vi "ReversedEngineering CreateStateTransationEdges.vi"(1 "GraphRefToAddNodesTo":refnum<class "Graph.lvclass">, 2 "StateDiagramReverseOptions":T1={"Clear All Current States"=TRUE, "UseMenuItem"=TRUE, "InsertArrayQueuedElementsVI"="", "Add Actions"=FALSE, "StateDiagramSerachActions"={"Action"=enum."NotTheseVIs", "VINames"=[], "LimitActions(VIs)"=10}, "AddCaseCommentsAsActions"=FALSE, "IgnoreStatesNotUsed"=FALSE, "CommentsSerachActions"={"MinimumTextLength"=0, "OnlyTopLeftComment"=FALSE, "CommentPrefix"=""}, "TransitionMode"=enum."Add to current transtion text", "ActionMode"=enum."Add to current action text"}, 3 "States":T5[](array[typedef]), 5 "error in (no error)":errorcluster, 7 "graphics":refnum<class "Graphics.lvclass">, 9 "grid":refnum<class "Grid.lvclass">) -> (19 "error out":errorcluster)   [LabVIEW 2020]
uses:
  <resource>/Framework/Providers/Open_GDS/UML/ReversedEngineering/ReversedEngineering StateMachineStateInfo.ctl
  <resource>/Framework/Providers/Open_GDS/UML/Graph_class/Graph.lvclass
  <resource>/Framework/Providers/Open_GDS/UML/Graphics_class/Graphics.lvclass
  <resource>/Framework/Providers/Open_GDS/UML/Grid_class/Grid.lvclass
  <resource>/Framework/Providers/Open_GDS/UML/ReversedEngineering/private/ReversedEngineering StateDiagramReverseOptions.ctl
  <resource>/Framework/Providers/Open_GDS/UML/ReversedEngineering/private/ReversedEngineering StateDiagramSerachActions.ctl
  <resource>/Framework/Providers/Open_GDS/UML/ReversedEngineering/ReversedEngineering StateAnalyseVIAction.ctl
  <resource>/Framework/Providers/Open_GDS/UML/ReversedEngineering/private/ReversedEngineering StateDiagramCommentSearchType.ctl
  <resource>/Framework/Providers/Open_GDS/UML/AbstractEdge_class/AbstractEdge.lvclass
  <resource>/Framework/Providers/Open_GDS/UML/StateNode_class/StateNode.lvclass
  <resource>/Framework/Providers/Open_GDS/UML/StateTransitionEdge_class/StateTransitionEdge.lvclass
  C:/Program Files (x86)/National Instruments/LabVIEW 2020/resource/Framework/Providers/Open_GDS/UML/AbstractEdge_class/AbstractEdge.lvclass
  <resource>/Framework/Providers/Open_GDS/UML/MultiLineString_class/MultiLineString.lvclass
  <resource>/Framework/Providers/Open_GDS/UML/AbstractNode_class/AbstractNode.lvclass
  <resource>/Framework/Providers/Open_GDS/UML/StateReverse_class/StateReverse.lvclass
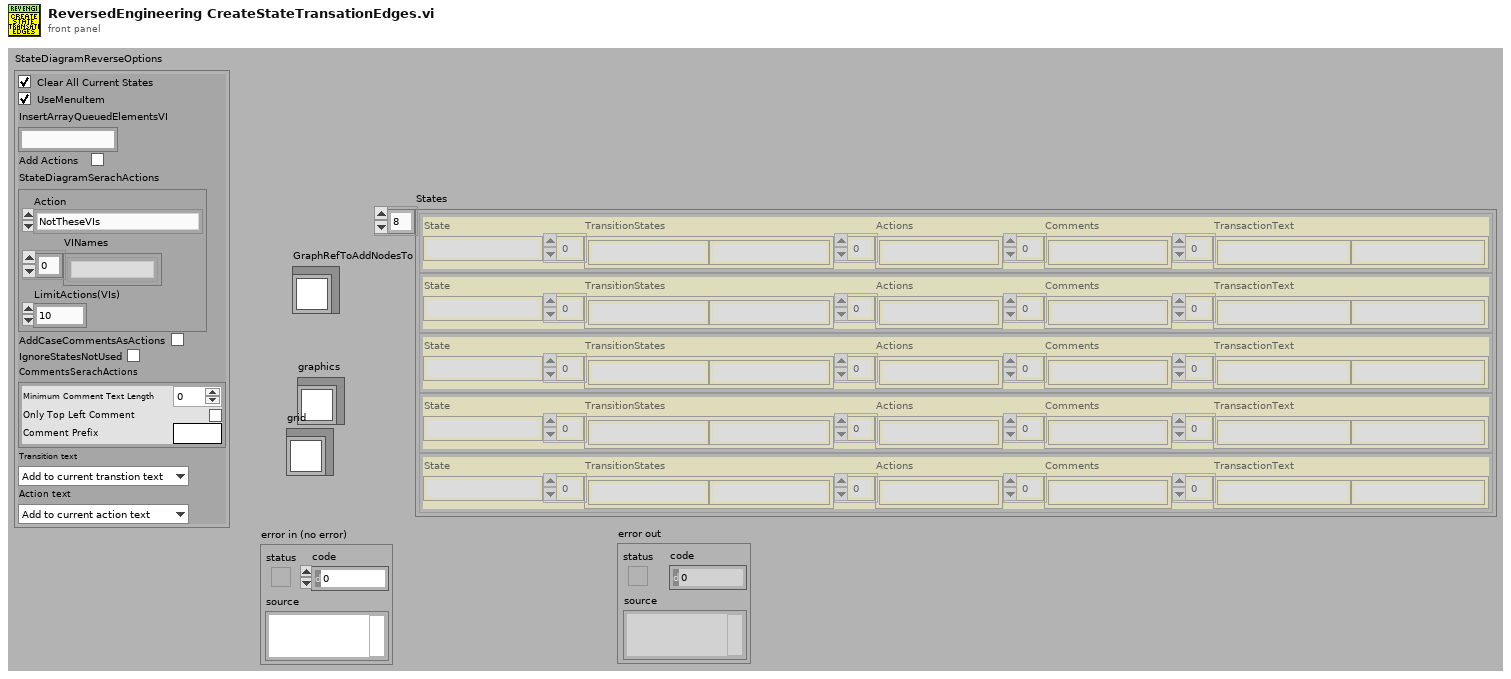
[diagram p1: front panel]
types:
  T1 = typedef "ReversedEngineering StateDiagramReverseOptions.ctl" = cluster{"Clear All Current States":bool, "UseMenuItem":bool, "InsertArrayQueuedElementsVI":string, "Add Actions":bool, "StateDiagramSerachActions":T2, "AddCaseCommentsAsActions":bool, "IgnoreStatesNotUsed":bool, "CommentsSerachActions":T4, "TransitionMode":enum16{"Add to current transtion text", "Replace transition text"}, "ActionMode":enum16{"Add to current action text", "Replace action text"}}
  T2 = typedef "ReversedEngineering StateDiagramSerachActions.ctl" = cluster{"Action":T3, "VINames":string[], "LimitActions(VIs)":i32}
  T3 = typedef "ReversedEngineering StateAnalyseVIAction.ctl" = enum16{"OnlyTheseVIs", "NotTheseVIs"}
  T4 = typedef "ReversedEngineering StateDiagramCommentSearchType.ctl" = cluster{"MinimumTextLength":i32, "OnlyTopLeftComment":bool, "CommentPrefix":string}
  T5 = typedef "ReversedEngineering StateMachineStateInfo.ctl" = cluster{"State":string, "TransitionStates":string[], "Actions":string[], "Comments":string[], "TransactionText":string[]}
  T6 = enum16{"Add to current transtion text", "Replace transition text"}
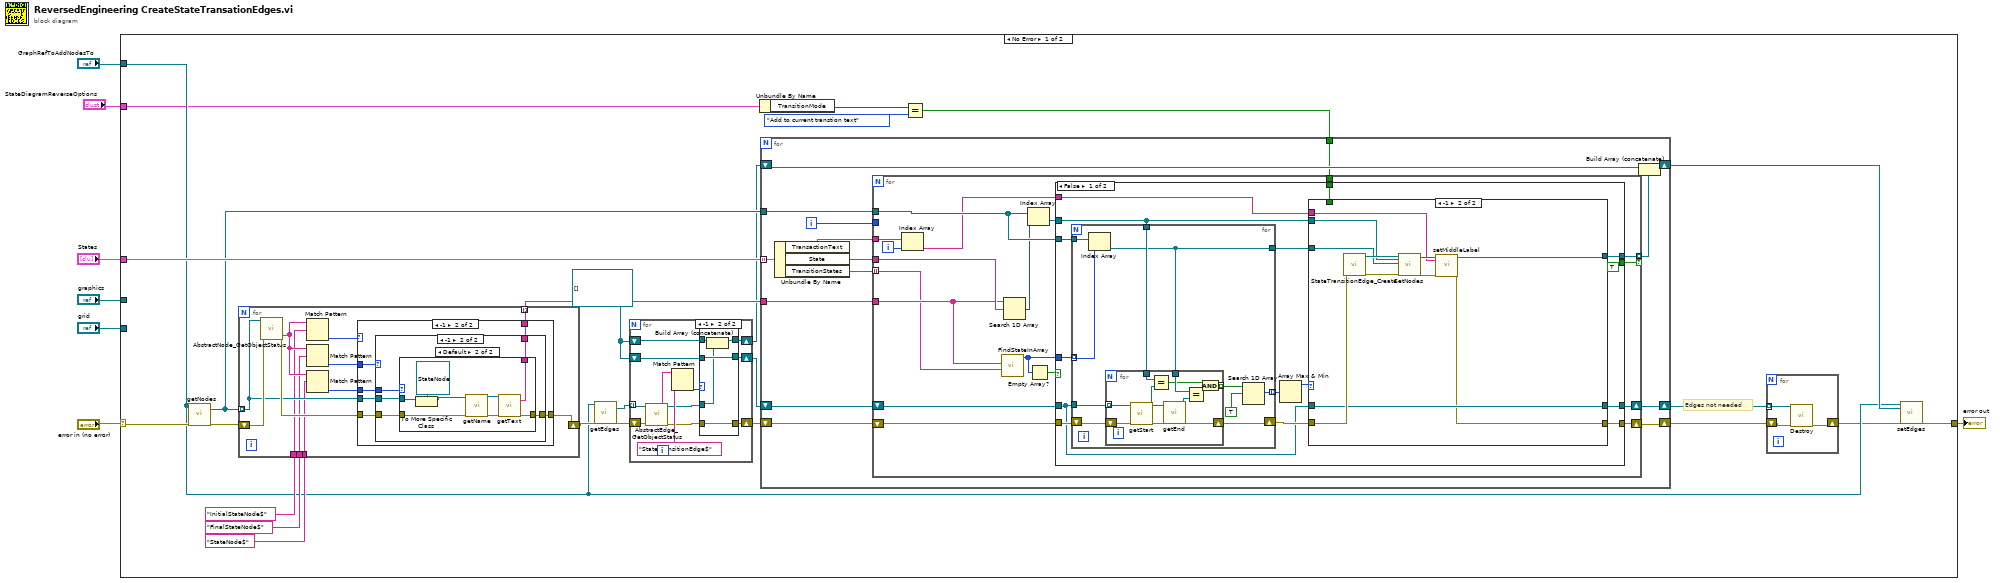
[diagram p0: block diagram]
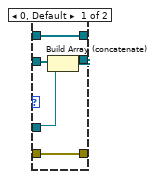
[diagram p2: hidden frame]
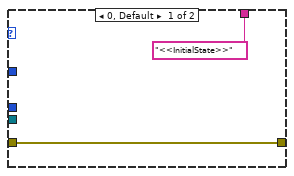
[diagram p3: hidden frame]
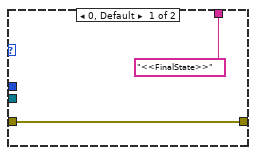
[diagram p4: hidden frame]
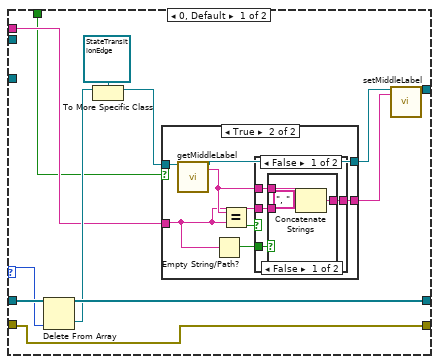
[diagram p6: hidden frame]
diagram:
  n1 = case shown="No Error" "error in (no error)" {
    selector: "error in (no error)" -> [w32 w208]
    tunnel: [w31 w208] -> w6
    tunnel: "States" -> [w30 _]
    tunnel: "GraphRefToAddNodesTo" -> [w21 _]
    tunnel: "graphics" -> [_ _]
    tunnel: "grid" -> [_ _]
    tunnel: "StateDiagramReverseOptions" -> [w11 _]
    frame No Error {
      w13 = refnum<class "AbstractEdge.lvclass">[] []
      # "Edges not needed"
      n2 = call-dynamic "getNodes.vi"("reference"=w21, "error in (no error)"=w32) -> ("nodes"=w29:refnum<class "AbstractNode.lvclass">[], "error out"=w24:errorcluster)  [unwired: 15 in, 1 out]
      n3 = for {
        shift-right: [w66] -> w22
        shift-left: w24 -> [w67]
        tunnel: w29 -> [w64] mode=indexing
        tunnel: [w65] -> w28 mode=indexing
        tunnel: "StateNode$" -> [w63]
        tunnel: "FinalStateNode$" -> [w61]
        tunnel: "InitialStateNode$" -> [w60]
        n4 = call <resource>:"AbstractNode_GetObjectStatus.vi"("reference in"=w64, "error in (no error)"=w67) -> ("Class name"=w62:string, "error out"=w69:errorcluster)  [unwired: 16 out]
        n5 = Match Pattern(string=w62, regular expression=w60) -> (offset past match=w59:i32)  [unwired: 4 out]
        n6 = Match Pattern(string=w62, regular expression=w61) -> (offset past match=w58:i32)  [unwired: 4 out]
        n7 = Match Pattern(string=w62, regular expression=w63) -> (offset past match=w68:i32)  [unwired: 4 out]
        n8 = case shown="-1" w59 {
          tunnel: w69 -> [w70 w77]
          tunnel: w68 -> [_ w76]
          tunnel: [w70 w75] -> w66
          tunnel: ["<<InitialState>>" ("text") w74] -> w65
          tunnel: w64 -> [_ w73]
          tunnel: w58 -> [_ w72]
          frame 0, Default {
          }
          frame -1 {
            n9 = case shown="-1" w72 {
              tunnel: w77 -> [w78 w84]
              tunnel: w76 -> [_ w83]
              tunnel: [w78 w82] -> w75
              tunnel: ["<<FinalState>>" ("text") w81] -> w74
              tunnel: w73 -> [_ w80]
              frame 0, Default {
              }
              frame -1 {
                n10 = case shown="Default" w83 {
                  tunnel: w80 -> [_ w88]
                  tunnel: w84 -> [w85 w93]
                  tunnel: [w85 w90] -> w82
                  tunnel: [_ w89] -> w81
                  frame -1 {
                  }
                  frame Default {
                    n11 = To More Specific Class(target class=refnum<class "StateNode.lvclass"> refnum ("reference"), reference=w88) -> (specific class reference=w86:refnum<class "StateNode.lvclass">)  [unwired: 1 in, 1 out]
                    n12 = call-dynamic "getName.vi"("reference"=w86, "error in (no error)"=w93) -> ("name"=w92:refnum<class "MultiLineString.lvclass">, "error out"=w91:errorcluster)  [unwired: 15 in, 1 out]
                    n13 = call-dynamic "getText.vi"("reference"=w92, "error in (no error)"=w91) -> ("text"=w89:string, "error out"=w90:errorcluster)  [unwired: 15 in, 1 out]
                  }
                }
              }
            }
          }
        }
      }
      n14 = call-dynamic "getEdges.vi"("reference"=w21, "error in (no error)"=w22) -> ("edges"=w16:refnum<class "AbstractEdge.lvclass">[], "error out"=w17:errorcluster)  [unwired: 15 in, 1 out]
      n15 = for {
        tunnel: w16 -> [w44] mode=indexing
        shift-right: [w39] -> w14
        shift-left: w17 -> [w43]
        shift-right: [w35] -> w15
        shift-left: w13 -> [w36]
        shift-right: [w33] -> w12
        shift-left: w13 -> [w34]
        n16 = call <resource>:"AbstractEdge_GetObjectStatus.vi"("reference in"=w44, "error in (no error)"=w43) -> ("Class name"=w42:string, "reference out"=w38:refnum<class "AbstractEdge.lvclass">, "error out"=w40:errorcluster)  [unwired: 15 out]
        n17 = Match Pattern(string=w42, regular expression="StateTransitionEdge$") -> (offset past match=w37:i32)  [unwired: 4 out]
        n18 = case shown="-1" w37 {
          tunnel: w40 -> [w49 w53]
          tunnel: [w49 w53] -> w39
          tunnel: w38 -> [w46 w50]
          tunnel: w36 -> [w48 w54]
          tunnel: [w47 w54] -> w35
          tunnel: w34 -> [w45 w52]
          tunnel: [w45 w51] -> w33
          frame 0, Default {
            n19 = Build Array (concatenate)(w48, w46) -> (w47:refnum<class "AbstractEdge.lvclass">[])
          }
          frame -1 {
            n20 = Build Array (concatenate)(w52, w50) -> (w51:refnum<class "AbstractEdge.lvclass">[])
          }
        }
      }
      n21 = Unbundle By Name(w11) -> ("TransitionMode"=w10:T6)
      n22 = Equal?(x=w10, y=T6."Add to current transtion text") -> (x = y?=w8:bool)
      n23 = for {
        shift-right: [w105] -> w20
        shift-left: w14 -> [w106]
        tunnel: w30 -> [w108] mode=indexing
        tunnel: w29 -> [w104]
        shift-right: [w102] -> w23
        shift-left: w12 -> [w100]
        tunnel: w28 -> [w98]
        shift-right: [w96] -> w19
        shift-left: w15 -> [w97]
        tunnel: w8 -> [w94]
        i -> [w99]
        n24 = Unbundle By Name(w108) -> ("TransactionText"=w95:string[], "State"=w107:string, "TransitionStates"=w103:string[])
        n25 = for {
          tunnel: w107 -> [w123]
          shift-right: [w126] -> w105
          shift-left: w106 -> [w118]
          tunnel: w104 -> [w125]
          tunnel: w103 -> [w116] mode=indexing
          tunnel: [w124] -> w101 mode=indexing if=w109
          tunnel: w99 -> [_]
          tunnel: w98 -> [w117]
          shift-right: [w120] -> w96
          shift-left: w97 -> [w119]
          tunnel: w95 -> [w115]
          tunnel: w94 -> [w112]
          i -> [w114]
          n26 = Index Array(array=w115, index=w114) -> (element=w113:string)
          n27 = call <resource>:"FindStateInArray.vi"("TransactionState"=w116, "AllCaseStates"=w117) -> ("AllIndexes"=w111:i32[])  [unwired: 7 in, 2 out]
          n28 = Search 1D Array(1D array=w117, element=w123) -> (index of element=w122:i32)  [unwired: 1 out]
          n29 = Index Array(array=w125, index=w122) -> (element=w121:refnum<class "AbstractNode.lvclass">)
          n30 = Empty Array?(array=w111) -> (empty?=w110:bool)
          n31 = case shown="False" w110 {
            tunnel: [w141 w206] -> w126
            tunnel: w125 -> [w140 _]
            tunnel: [w139 _] -> w124
            tunnel: w121 -> [w138 _]
            tunnel: [w136 w207] -> w120
            tunnel: w119 -> [w127 w207]
            tunnel: w118 -> [w133 w206]
            tunnel: w113 -> [w131 _]
            tunnel: w112 -> [w130 _]
            tunnel: w111 -> [w129 _]
            tunnel: [TRUE _] -> w109
            frame False {
              n32 = for {
                tunnel: w140 -> [w151]
                tunnel: w138 -> [w150]
                tunnel: [w149] -> w137
                tunnel: [w146] -> w135 mode=indexing
                tunnel: w127 -> [w145]
                shift-right: [w144] -> w132
                shift-left: w133 -> [w143]
                tunnel: w129 -> [w142] mode=indexing
                n33 = Index Array(array=w151, index=w142) -> (element=w149:refnum<class "AbstractNode.lvclass">)
                n34 = for {
                  shift-right: [w153] -> w144
                  shift-left: w143 -> [w162]
                  tunnel: w145 -> [w161] mode=indexing
                  tunnel: w150 -> [w159]
                  tunnel: w149 -> [w156]
                  tunnel: [w152] -> w148 mode=indexing
                  n35 = call-dynamic "getStart.vi"("reference"=w161, "error in (no error)"=w162) -> ("reference out"=w160:refnum<class "AbstractEdge.lvclass">, "startNode"=w158:refnum<class "AbstractNode.lvclass">, "error out"=w163:errorcluster)  [unwired: 14 in, 1 out]
                  n36 = Equal?(x=w159, y=w158) -> (x = y?=w155:bool)
                  n37 = call-dynamic "getEnd.vi"("reference"=w160, "error in (no error)"=w163) -> ("endNode"=w157:refnum<class "AbstractNode.lvclass">, "error out"=w153:errorcluster)  [unwired: 14 in, 2 out]
                  n38 = Equal?(x=w156, y=w157) -> (x = y?=w154:bool)
                  n39 = And(x=w155, y=w154) -> (x .and. y?=w152:bool)
                }
                n40 = Search 1D Array(1D array=w148, element=TRUE) -> (index of element=w146:i32)  [unwired: 1 out]
              }
              n41 = Array Max & Min(array=w135) -> (max value=w134:i32)  [unwired: 3 out]
              n42 = case shown="-1" w134 {
                selector: w134 -> [w174 _]
                tunnel: [w172 w196] -> w141
                tunnel: [w169 w198] -> w139
                tunnel: w138 -> [_ w203]
                tunnel: w137 -> [_ w202]
                tunnel: w132 -> [w172 w201]
                tunnel: w127 -> [w175 w200]
                tunnel: [w173 w200] -> w136
                tunnel: w131 -> [w166 w195]
                tunnel: w130 -> [w164 _]
                frame 0, Default {
                  n43 = Delete From Array(array=w175, index=w174) -> (deleted portion=w170:refnum<class "AbstractEdge.lvclass">, array with subset deleted=w173:refnum<class "AbstractEdge.lvclass">[])  [unwired: 1 in]
                  n44 = To More Specific Class(target class=refnum<class "StateTransitionEdge.lvclass"> refnum ("reference"), reference=w170) -> (specific class reference=w168:refnum<class "StateTransitionEdge.lvclass">)  [unwired: 1 in, 1 out]
                  n45 = case shown="True" w164 {
                    tunnel: w168 -> [w176 w183]
                    tunnel: [w176 w182] -> w167
                    tunnel: [w177 w184] -> w165
                    tunnel: w166 -> [w177 w179]
                    frame False {
                    }
                    frame True {
                      n46 = call-dynamic "getMiddleLabel.vi"("reference"=w183) -> ("reference out"=w182:refnum<class "StateTransitionEdge.lvclass">, "label"=w181:string)  [unwired: 16 in, 1 out]
                      n47 = Empty String/Path?(string/path=w179) -> (empty?=w178:bool)
                      n48 = Equal?(x=w181, y=w179) -> (x = y?=w180:bool)
                      n49 = case shown="False" w180 {
                        tunnel: [w188 w194] -> w184
                        tunnel: w181 -> [w187 _]
                        tunnel: w179 -> [w186 w194]
                        tunnel: w178 -> [w185 _]
                        frame False {
                          n50 = case shown="False" w185 {
                            tunnel: [w191 w193] -> w188
                            tunnel: w187 -> [w190 w193]
                            tunnel: w186 -> [w189 _]
                            frame False {
                              n51 = Concatenate Strings(w190, ", " ("string"), w189) -> (w191:string)
                            }
                            frame True {
                            }
                          }
                        }
                        frame True {
                        }
                      }
                    }
                  }
                  n52 = call-dynamic "setMiddleLabel.vi"("reference"=w167, "middleLabel"=w165) -> ("reference out"=w169:refnum<class "StateTransitionEdge.lvclass">)  [unwired: 16 in, 1 out]
                }
                frame -1 {
                  n53 = call <resource>:"StateTransitionEdge_Create.vi"("error in (no error)"=w201) -> ("reference out"=w205:refnum<class "StateTransitionEdge.lvclass">, "error out"=w204:errorcluster)  [unwired: 1 in, 16 out]
                  n54 = call-dynamic "SetNodes.vi"("reference"=w205, "Start"=w203, "End"=w202, "error in (no error)"=w204) -> ("reference out"=w199:refnum<class "StateTransitionEdge.lvclass">, "error out"=w197:errorcluster)  [unwired: 14 in]
                  n55 = call-dynamic "setMiddleLabel.vi"("reference"=w199, "middleLabel"=w195, "error in (no error)"=w197) -> ("reference out"=w198:refnum<class "StateTransitionEdge.lvclass">, "error out"=w196:errorcluster)  [unwired: 15 in]
                }
              }
            }
            frame True {
            }
          }
        }
        n56 = Build Array (concatenate)(w100, w101) -> (w102:refnum<class "AbstractEdge.lvclass">[])
      }
      n57 = for {
        shift-right: [w55] -> w18
        shift-left: w20 -> [w57]
        tunnel: w19 -> [w56] mode=indexing
        n58 = call-dynamic "Destroy.vi"("reference"=w56, "error in (no error)"=w57) -> ("error out"=w55:errorcluster)  [unwired: 17 in]
      }
      n59 = call-dynamic "setEdges.vi"("reference"=w21, "edges"=w23, "error in (no error)"=w18) -> ("error out"=w31:errorcluster)  [unwired: 15 in, 1 out]
    }
    frame Error {
    }
  }
  "error out" <- w6
